vi "delete mapping by channel.vi"(7 "owner ID":string, 8 "error in":errorcluster, 10 "channel":refnum<class "TBM channel.lvclass">, 11 "engine configuration in":refnum<class "engine configuration.lvclass">) -> (0 "error out":errorcluster, 3 "engine configuration out":refnum<class "engine configuration.lvclass">)   [LabVIEW 2014, in "engine configuration.lvclass"]
doc: "This function deletes the mapping associated with a specific module and channel."
uses:
  engine configuration.lvclass
  <vilib>/NI/Tag Bus Module Framework/channel/TBM channel.lvclass
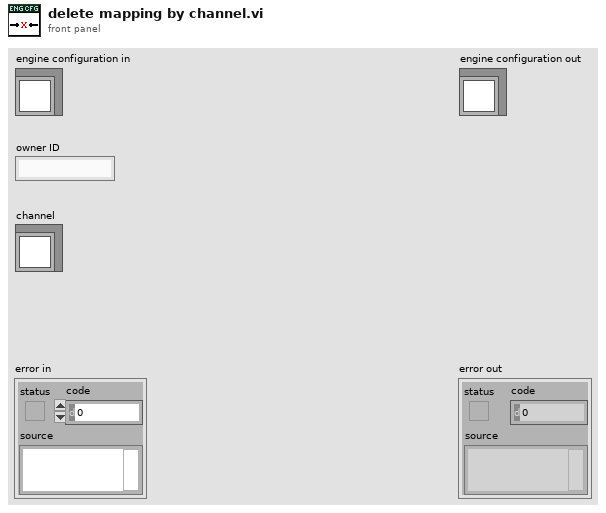
[diagram p1: front panel]
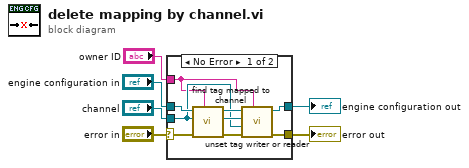
[diagram p0: block diagram]
diagram:
  n1 = case shown="No Error" "error in" {
    selector: "error in" -> [w11 w17]
    tunnel: [w15 w17] -> w5
    tunnel: [w14 w16] -> w3
    tunnel: "engine configuration in" -> [w13 w16]
    tunnel: "owner ID" -> [w7 _]
    tunnel: "channel" -> [w8 _]
    frame No Error {
      n2 = call "find tag mapped to channel.vi"("owner"=w7, "error in"=w11, "channel"=w8, "engine configuration in"=w13) -> ("error out"=w10:errorcluster, "tag"=w9:refnum<class "tag descriptor.lvclass">, "engine configuration out"=w12:refnum<class "engine configuration.lvclass">)  [unwired: 5 in]
      n3 = call-dynamic "unset tag writer or reader.vi"("module GUID"=w7, "error in"=w10, "channel"=w8, "tag descriptor"=w9, "engine configuration in"=w12) -> ("error out"=w15:errorcluster, "engine configuration out"=w14:refnum<class "engine configuration.lvclass">)  [unwired: 5 in]
    }
    frame Error {
    }
  }
  "error out" <- w5
  "engine configuration out" <- w3
